vi "subDetermineNeedRebuildingFromHashes.vi"(8 "Force rebuild":bool, 9 "Dependency files":set{path}(c389), 10 "ProjectItem in":refnum<class "ProjectItem.lvclass">, 11 "Hashes in":T1) -> (1 "Needs rebuilding":bool, 2 "Log string":string, 3 "Hashes out":T1)   [LabVIEW 2019, in "SolutionBuilder.lvlib" / "SolutionBuilder.lvclass"]
uses:
  SolutionBuilder.lvclass
  Hashes.ctl
  HashMap.ctl
  Community/SolutionProjectInfo.ctl
  ProjectItem/ProjectItem.lvclass
  ProjectItem/ProjectItem.lvclass/ProjectItem.ctl
  <vilib>/Utility/miscctls.llb/LVMapReplaceAction.ctl
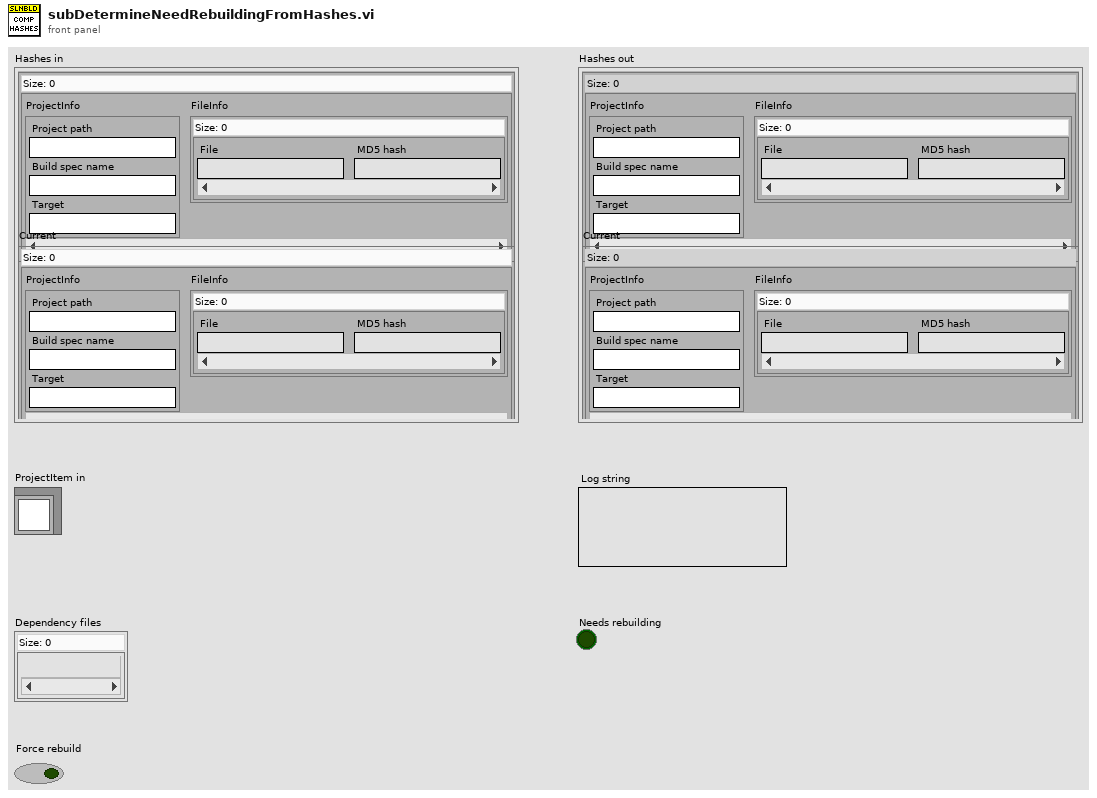
[diagram p1: front panel]
types:
  T1 = typedef "SolutionBuilder.lvlib/SolutionBuilder.lvclass/Hashes.ctl" = cluster{"Previous":T2, "Current":T2}
  T2 = typedef "SolutionBuilder.lvlib/SolutionBuilder.lvclass/HashMap.ctl" = map{T3, map{string, string}}
  T3 = typedef "SolutionBuilder.lvlib/SolutionBuilder.lvclass/SolutionProjectInfo.ctl" = cluster{"Project path":string, "Build spec name":string, "Target":string}
  T4 = typedef "LVMapReplaceAction.ctl" = enum32{"Modify Entry only if found", "Add or Modify Entry", "Delete Entry"}
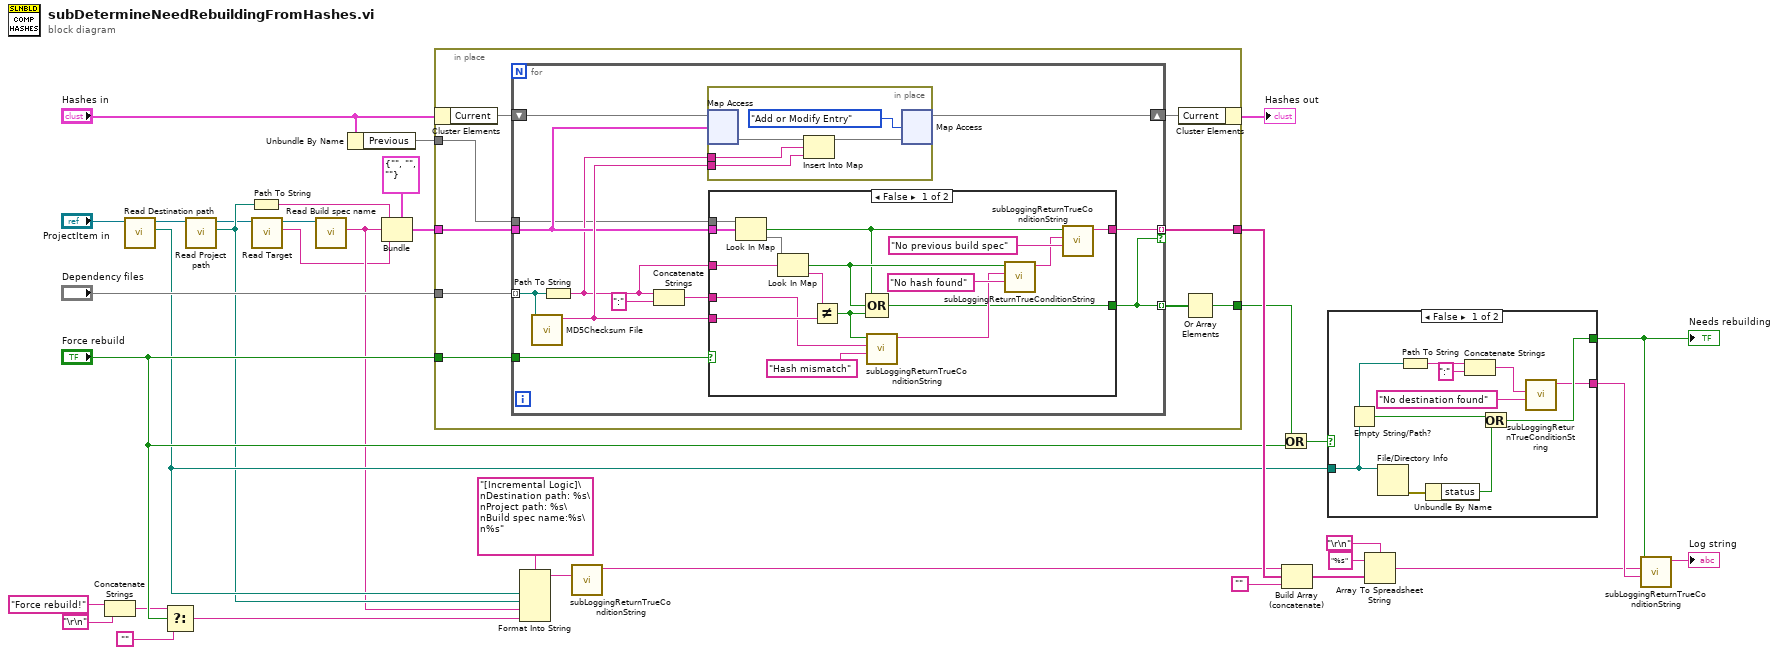
[diagram p0: block diagram]
diagram:
  n1 = Concatenate Strings("Force rebuild!" ("True string"), "\r\n") -> (w12:string)
  n2 = call "Read Destination path.vi"("ProjectItem in"="ProjectItem in") -> ("Destination path"=w9:path, "ProjectItem out"=w29:refnum<class "ProjectItem.lvclass">)  [unwired: 9 in]
  n3 = Select(t=w12, s="Force rebuild", f="") -> (s? t:f=w6:string)
  n4 = call "Read Project path.vi"("ProjectItem in"=w29) -> ("Project path"=w8:path, "ProjectItem out"=w3:refnum<class "ProjectItem.lvclass">)  [unwired: 9 in]
  n5 = Path To String(path=w8) -> (string=w31:string)
  n6 = call "Read Target.vi"("ProjectItem in"=w3) -> ("Target"=w1:string, "ProjectItem out"=w2:refnum<class "ProjectItem.lvclass">)  [unwired: 9 in]
  n7 = call "Read Build spec name.vi"("ProjectItem in"=w2) -> ("Build spec name"=w7:string)  [unwired: 9 in, 1 out]
  n8 = Unbundle By Name("Hashes in") -> ("Previous"=w18:T2)
  n9 = Bundle(cluster=T3 {"Project path"="", "Build spec name"="", "Target"=""} ("key"), "Project path"=w31, "Build spec name"=w7, "Target"=w1) -> (w30:T3)
  n10 = in-place {
    in-place-border: "Dependency files" -> [w44]
    in-place-border: w30 -> [w43]
    in-place-border: [w42] -> w26
    in-place-border: w18 -> [w39]
    in-place-border: "Force rebuild" -> [w38]
    in-place-border: [w36] -> w16
    n11 = in-place-cluster #1("Hashes in") -> ("Current"=w41:T2)
    n12 = for {
      shift-right: [w53] -> w40
      shift-left: w41 -> [w55]
      tunnel: w44 -> [w56] mode=indexing
      tunnel: [w47] -> w37 mode=indexing
      tunnel: w43 -> [w52]
      tunnel: [w48] -> w42 mode=indexing if=w47
      tunnel: w39 -> [w46]
      tunnel: w38 -> [w45]
      n13 = call <vilib>:"MD5Checksum File.vi"("Path"=w56) -> ("MD5 message-digest"=w54:string)  [unwired: 9 in, 1 out]
      n14 = Path To String(path=w56) -> (string=w51:string)
      n15 = Concatenate Strings(w51, ":" ("string")) -> (w49:string)
      n16 = in-place {
        in-place-border: w51 -> [w58]
        in-place-border: w54 -> [w57]
        n17 = in-place-map #2(w55, w52) -> (w61:map{string, string})  [unwired: 1 in, 1 out]
        n18 = Insert Into Map(map in=w61, key=w58, value=w57) -> (map out=w60:map{string, string})  [unwired: 2 out]
        n19 = in-place-map #2(w60, LVMapReplaceAction."Add or Modify Entry" ("action")) -> (w53:T2)  [unwired: 2 out]
      }
      n20 = case shown="False" w45 {
        tunnel: w46 -> [w78 _]
        tunnel: w54 -> [w75 _]
        tunnel: w52 -> [w74 _]
        tunnel: w51 -> [w67 _]
        tunnel: w49 -> [w66 _]
        tunnel: [w63 _] -> w48
        tunnel: [w62 _] -> w47
        frame False {
          n21 = Look In Map(map=w78, key=w74) -> (key not found?=w68:bool, value=w77:map{string, string})  [unwired: 1 in]
          n22 = Look In Map(map=w77, key=w67) -> (key not found?=w71:bool, value=w76:string)  [unwired: 1 in]
          n23 = Not Equal?(x=w76, y=w75) -> (x != y?=w72:bool)
          n24 = Compound Arithmetic op=OR(w68, w71, w72) -> (w62:bool)
          n25 = call "subLoggingReturnTrueConditionString.vi"("True string"="Hash mismatch" ("t"), "Initial string"=w66, "Condition (T)"=w72) -> ("Log string"=w65:string)  [unwired: 8 in]
          n26 = call "subLoggingReturnTrueConditionString.vi"("True string"="No hash found", "Initial string"=w65, "Condition (T)"=w71) -> ("Log string"=w64:string)  [unwired: 8 in]
          n27 = call "subLoggingReturnTrueConditionString.vi"("True string"="No previous build spec", "Initial string"=w64, "Condition (T)"=w68) -> ("Log string"=w63:string)  [unwired: 8 in]
        }
        frame True {
        }
      }
    }
    n28 = in-place-cluster #1("Current"=w40) -> (→"Hashes out":T1)
    n29 = Or Array Elements(Boolean array=w37) -> (logical OR=w36:bool)
  }
  n30 = Format Into String(format string="[Incremental Logic]\nDestination path: %s\nProject path: %s\nBuild spec name:%s\n%s", w9, w8, w7, w6) -> (resulting string=w5:string)  [unwired: 2 in, 1 out]
  n31 = call "subLoggingReturnTrueConditionString.vi"("Initial string"=w5) -> ("Log string"=w25:string)  [unwired: 10 in]
  n32 = Or(x=w16, y="Force rebuild") -> (x .or. y?=w15:bool)
  n33 = Build Array (concatenate)(w25, w26, "") -> (w24:string[])
  n34 = case shown="False" w15 {
    selector: w15 -> [_ w89]
    tunnel: [w85 w89] -> w20
    tunnel: w9 -> [w80 _]
    tunnel: [w83 _] -> w23
    frame False {
      n35 = Empty String/Path?(string/path=w80) -> (empty?=w87:bool)
      n36 = File/Directory Info(path=w80) -> (error out=w88:errorcluster)  [unwired: 1 in, 6 out]
      n37 = Path To String(path=w80) -> (string=w82:string)
      n38 = Unbundle By Name(w88) -> ("status"=w86:bool)
      n39 = Concatenate Strings(w82, ":" ("string")) -> (w79:string)
      n40 = Or(x=w87, y=w86) -> (x .or. y?=w85:bool)
      n41 = call "subLoggingReturnTrueConditionString.vi"("True string"="No destination found" ("String"), "Initial string"=w79) -> ("Log string"=w83:string)  [unwired: 9 in]
    }
    frame True {
    }
  }
  "Needs rebuilding" <- w20
  n42 = Array To Spreadsheet String(delimiter (Tab)="\r\n", array=w24, 3:"%s" ("format string")) -> (spreadsheet string=w22:string)
  n43 = call "subLoggingReturnTrueConditionString.vi"("True string"=w23, "Initial string"=w22, "Condition (T)"=w20) -> ("Log string"=→"Log string":string)  [unwired: 8 in]
